vi "Measurement Logic.vi"() -> ()   [LabVIEW 2022 SP3, in "Stepped Frequency Sweep_Class D Amplifier.lvlib"]
uses:
  Stepped Frequency Sweep_Class D Amplifier.lvlib
  Measurement Results.ctl
  <vilib>/Analysis/NI_AALBase.lvlib
  <vilib>/Analysis/1siggen.llb/Ramp Pattern by Samples.vi
  <vilib>/Plug-In SDKs/Measurements/Measure Call Context/Measure Call Context.lvclass
  Measurement Configuration.ctl
  shared/controls/single tone audio measurements.ctl
  shared/controls/audio controls.lvlib
  shared/controls/weighting filter.ctl
  shared/controls/lowpass filter.ctl
  shared/controls/highpass filter.ctl
  shared/controls/sweep profile.ctl
  shared/controls/units - snr.ctl
  shared/controls/units - ratio.ctl
  shared/controls/digital output level units.ctl
  shared/controls/regulation target.ctl
  shared/controls/regulation target value units.ctl
panel:
  out "results":T1={"channel"="0", "frequency (Hz)"=1000.0000024177915, "amplitude (Vrms)"=-6.256665451281146, "amplitude (dBFS)"=78.42395339546047, "phase (deg)"=0.0, "SNR"=-71.07176133726693, "THD+N"=-71.98384642729017, "THD"=-0.25666545128114626, "dynamic range (dB)"=83.34902670182771, "gain"=102.93430172121762, "SFDR (dBc)"=0.0}
  out "Spectrum":cluster{"x0":dbl, "dx":dbl, "magnitude":dbl[]}(graph)
  out "Waveform Graph":waveform(dbl)(graph)
  out "measure call context out":refnum<class "Measure Call Context.lvclass">
  in  "measure call context in":refnum<class "Measure Call Context.lvclass">
  out "measurement results":T2={"channel name"="0", "frequency (Hz)"=[], "amplitude (Vrms)"=[], "amplitude (dBFS)"=[], "SNR"=[], "THD+N"=[], "THD"=[], "dynamic range (dB)"=[], "gain"=[], "SFDR (dBc)"=[], "output power (W)"=[], "wfm - t0"=0.0, "wfm - dt"=1.9531249997269942e-05, "wfm - data"=array[12800 elements], "fft - f0"=0.0, "fft - df"=4.000000000559116, "fft - data"=array[6400 elements]}
  in  "measurement configuration":T3={"digital serial cfg file"="", "digital channel list"="7821\\PCMo 8", "master clock channel list"="7821\\PCMo 0", "output level"=-10.0, "output level units"=enum."dBFS", "output range (pk-pk)"=15.0, "load impedance"=4.0, "signal phase"=0.0, "acq sampling rate"=51200.0, "min measurement cycles"=20, "min measurement time (s)"=0.1, "min settling cycles"=0, "min settling time (s)"=0.005, "acq channel"="PXI1Slot4/ai0", "band start"=20.0, "band stop"=20000.0, "weighting filter"=enum."Linear", "highpass filter"=enum."DC", "lowpass filter"=enum."No filter", "sweep start frequency (Hz)"=20.0, "sweep stop frequency (Hz)"=20000.0, "number of steps"=10, "sweep profile"=enum."Logarithmic", "SNR units"=enum."dB", "THD+N units"=enum."dB", "THD units"=enum."dB", "gain units"=enum."dB", "enable regulation"=FALSE, "regulation target"=enum."THD+N Ratio", "regulation target value"=10.0, "regulation target value units"=enum."%", "regulation start level"=-1.0, "regulation stop level"=-10.0, "regulation number of steps"=2} {"min measurement cycles" format="%#_6p"; "sweep stop frequency (Hz)" format="%0.2f"; "acq sampling rate" format="%0.2f"}
  out "error out":errorcluster
  in  "error in":errorcluster
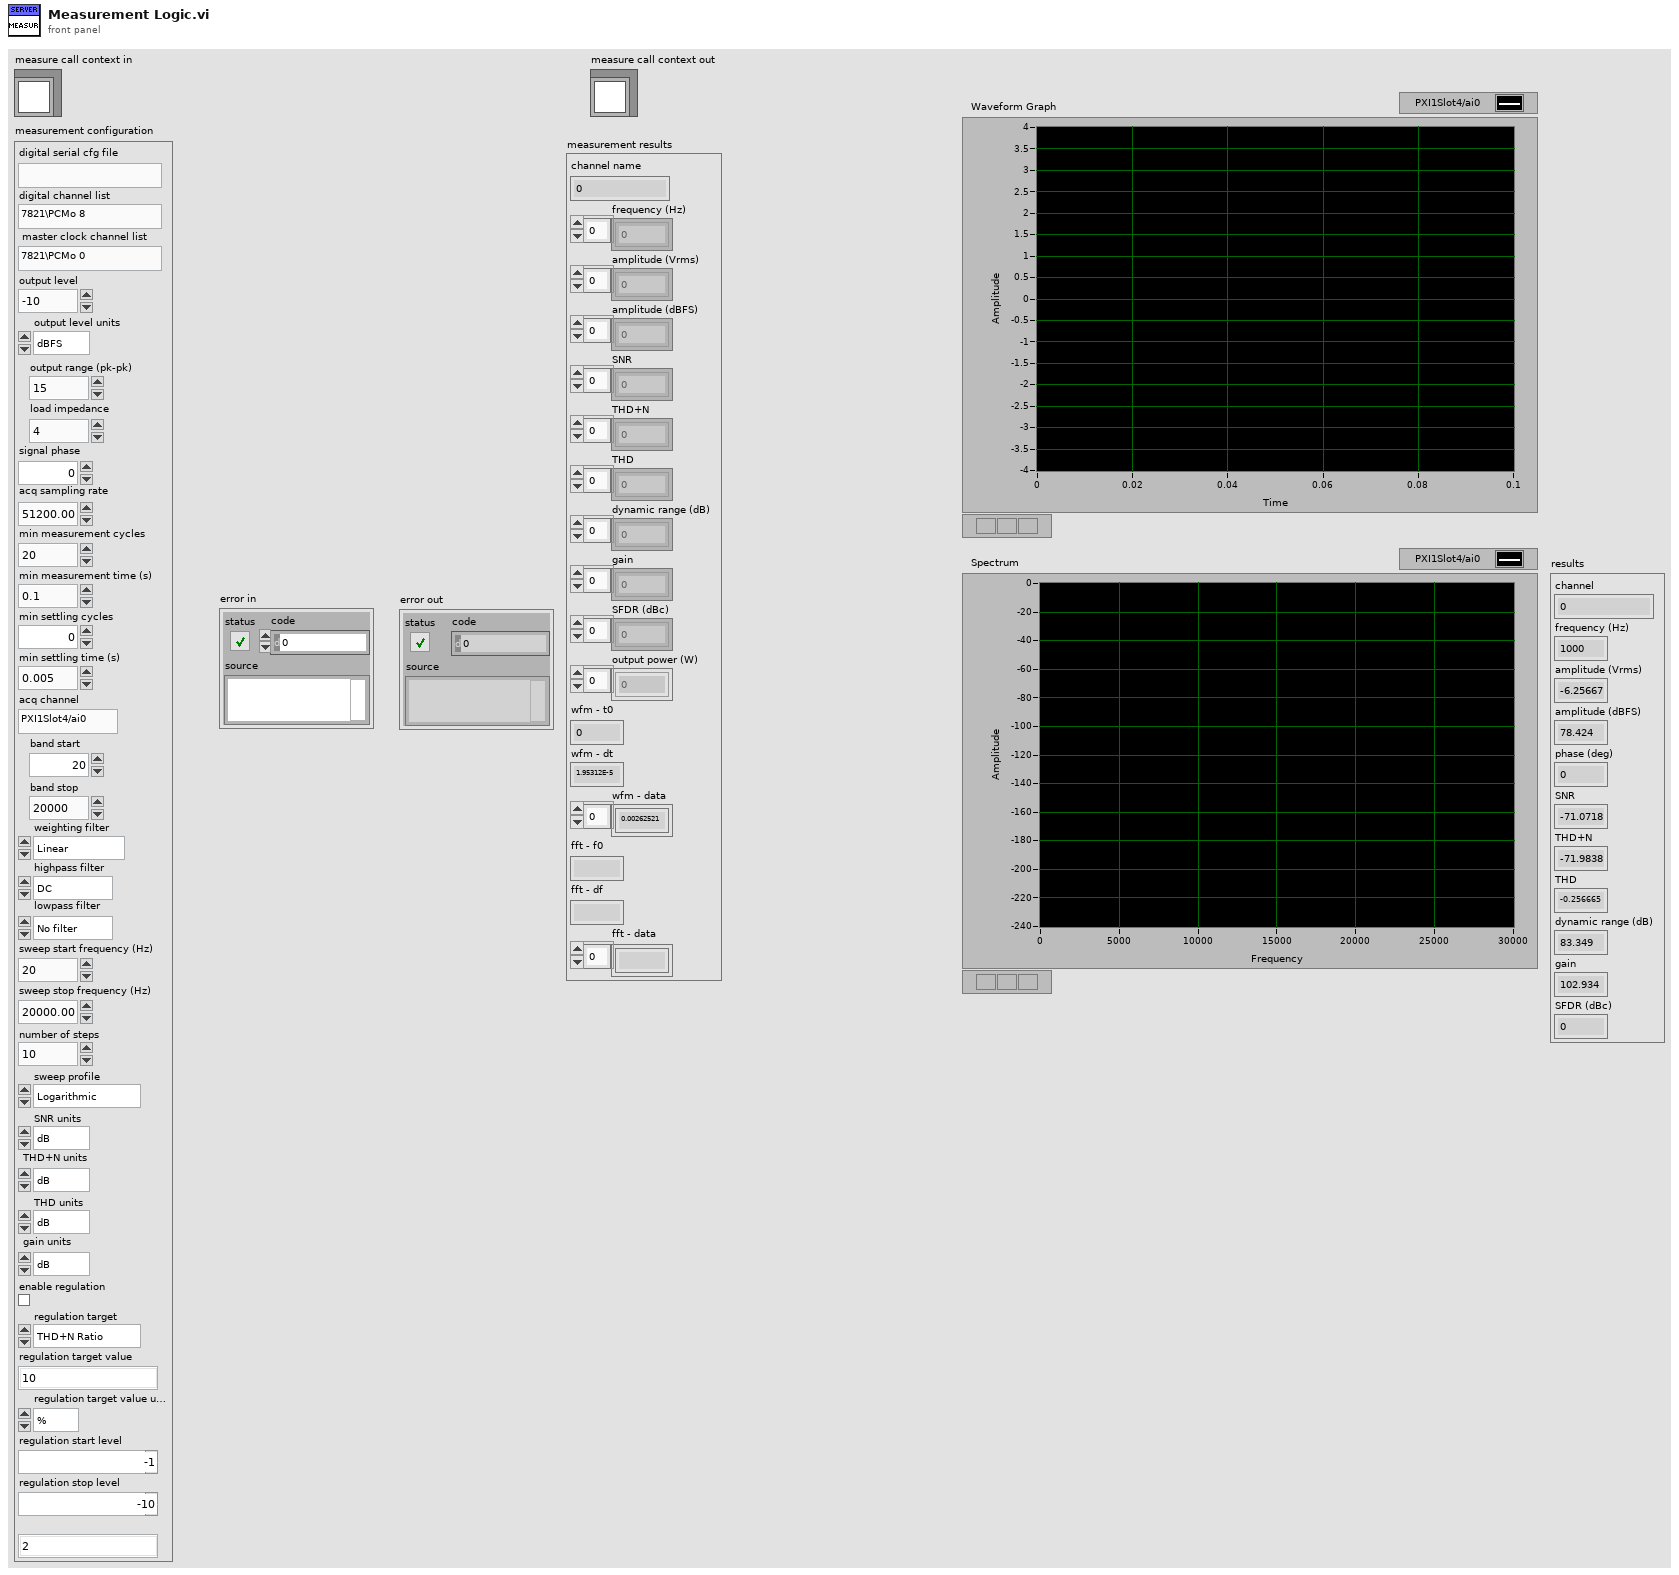
[diagram p1: front panel]
types:
  T1 = typedef "audio controls.lvlib/single tone audio measurements.ctl" = cluster{"channel":string, "frequency (Hz)":dbl, "amplitude (Vrms)":dbl, "amplitude (dBFS)":dbl, "phase (deg)":dbl, "SNR":dbl, "THD+N":dbl, "THD":dbl, "dynamic range (dB)":dbl, "gain":dbl, "SFDR (dBc)":dbl}
  T2 = typedef "Stepped Frequency Sweep_Class D Amplifier.lvlib/Measurement Results.ctl" = cluster{"channel name":string, "frequency (Hz)":dbl[], "amplitude (Vrms)":dbl[], "amplitude (dBFS)":dbl[], "SNR":dbl[], "THD+N":dbl[], "THD":dbl[], "dynamic range (dB)":dbl[], "gain":dbl[], "SFDR (dBc)":dbl[], "output power (W)":dbl[], "wfm - t0":dbl, "wfm - dt":dbl, "wfm - data":dbl[], "fft - f0":dbl, "fft - df":dbl, "fft - data":dbl[]}
  T3 = typedef "Stepped Frequency Sweep_Class D Amplifier.lvlib/Measurement Configuration.ctl" = cluster{"digital serial cfg file":string, "digital channel list":string, "master clock channel list":string, "output level":dbl, "output level units":T4, "output range (pk-pk)":dbl, "load impedance":dbl, "signal phase":dbl, "acq sampling rate":dbl, "min measurement cycles":u32, "min measurement time (s)":dbl, "min settling cycles":u32, "min settling time (s)":dbl, "acq channel":string, "band start":dbl, "band stop":dbl, "weighting filter":T5, "highpass filter":T6, "lowpass filter":T7, "sweep start frequency (Hz)":dbl, "sweep stop frequency (Hz)":dbl, "number of steps":u32, "sweep profile":T8, "SNR units":T9, "THD+N units":T10, "THD units":T10, "gain units":T10, "enable regulation":bool, "regulation target":T11, "regulation target value":dbl, "regulation target value units":T12, "regulation start level":dbl, "regulation stop level":dbl, "regulation number of steps":u32}
  T4 = typedef "audio controls.lvlib/digital output level units.ctl" = enum32{"% FS", "dBFS", "V"}
  T5 = typedef "weighting filter.ctl" = enum32{"Linear", "A-weighting", "B-weighting", "C-weighting"}
  T6 = typedef "highpass filter.ctl" = enum32{"DC", "AC"}
  T7 = typedef "lowpass filter.ctl" = enum32{"No filter", "AES17 20kHz", "AES17 40kHz"}
  T8 = typedef "audio controls.lvlib/sweep profile.ctl" = enum32{"Linear", "Logarithmic"}
  T9 = typedef "audio controls.lvlib/units - snr.ctl" = enum32{"dB", "x/y"}
  T10 = typedef "audio controls.lvlib/units - ratio.ctl" = enum32{"dB", "%", "x/y"}
  T11 = typedef "regulation target.ctl" = enum32{"THD+N Ratio", "Output Power"}
  T12 = typedef "regulation target value units.ctl" = enum32{"%", "W"}
  T13 = typedef "regulation settings.ctl" = cluster{"enable regulation":bool, "regulation target":T11, "regulation target value":dbl, "regulation target value units":T12, "regulation start level":dbl, "regulation stop level":dbl, "regulation number of steps":u32}
  T14 = typedef "single tone measurement settings (HW).ctl" = cluster{"digital channel list":string, "frame clock rate":dbl, "number of channels":u32, "channel length":u32, "bit depth":u32, "data justification":T15, "endianness":T16, "bit clock edge sync":T17, "frame sync edge for channel 0":T17, "channel 0 offset":u32, "master clock channel list":string, "master clock rate":dbl, "enable dither":bool, "logic level":T18, "signal frequency":dbl, "output level":dbl, "output level units":T4, "output range (pk-pk)":dbl, "load impedance":dbl, "signal phase":dbl, "acq sampling rate":dbl, "min measurement cycles":u32, "min measurement time (s)":dbl, "min settling cycles":u32, "min settling time (s)":dbl, "acq channel":string, "band start":dbl, "band stop":dbl, "weighting filter":T5, "highpass filter":T6, "lowpass filter":T7, "SNR units":T9, "THD+N units":T10, "THD units":T10, "gain units":T10}
  T15 = typedef "data justification.ctl" = enum32{"Left Justified", "Right Justified"}
  T16 = typedef "endianness.ctl" = enum32{"MSB First", "LSB First"}
  T17 = typedef "digital edge.ctl" = enum32{"Rising", "Falling"}
  T18 = typedef "logic level.ctl" = enum32{"3.3 V", "1.8 V", "1.2 V"}
  T19 = typedef "PCM tasks.ctl" = cluster{"PCM output task":T20, "PCM output task-clock":T20}
  T20 = typedef "PDM Acquisition Class Library.lvlib/PCM Output Task.lvclass/PCM Output Task DVR.ctl" = refnum<data-value>
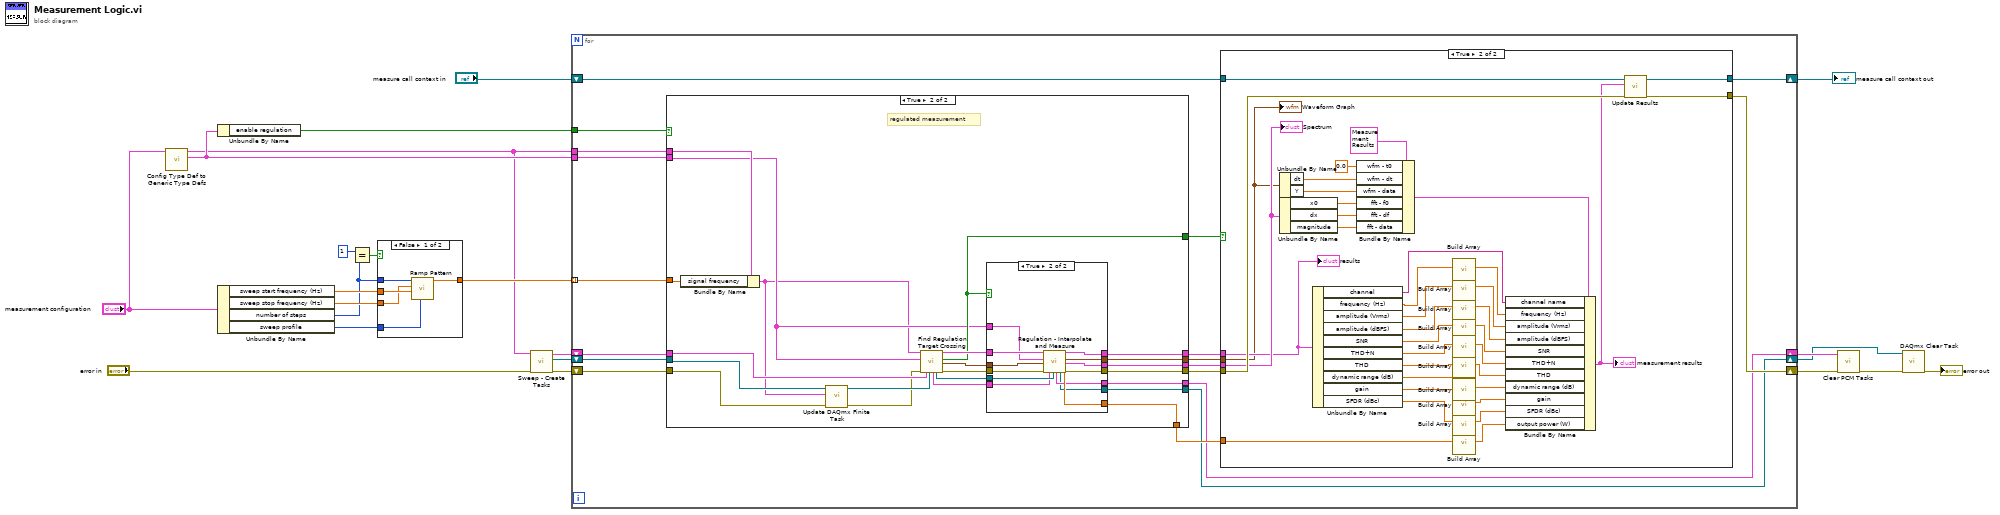
[diagram p0: block diagram]
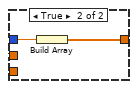
[diagram p2: hidden frame]
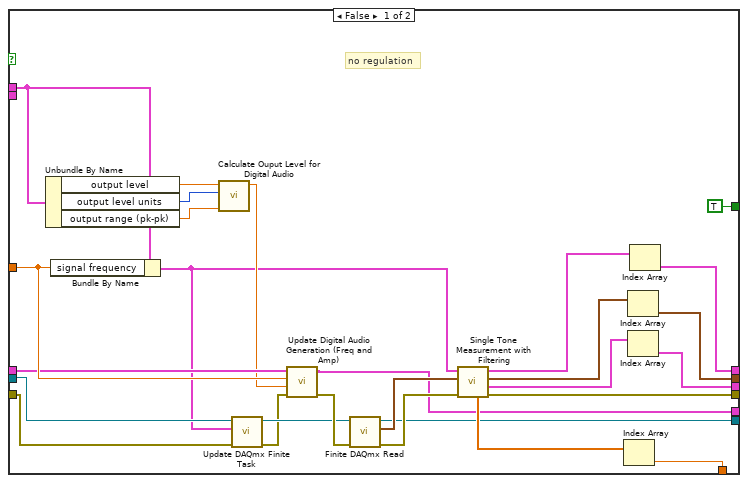
[diagram p4: hidden frame]
diagram:
  n1 = call "Config Type Def to Generic Type Defs.vi"("measurement configuration"="measurement configuration") -> ("regulation settings"=w11:T13, "single tone settings"=w8:T14)  [unwired: 9 in]
  n2 = Unbundle By Name(w11) -> ("enable regulation"=w13:bool)
  n3 = Unbundle By Name("measurement configuration") -> ("sweep start frequency (Hz)"=w21:dbl, "sweep stop frequency (Hz)"=w20:dbl, "number of steps"=w16:u32, "sweep profile"=w22:T8)
  n4 = Equal?(x=u32 1, y=w16) -> (x = y?=w17:bool)
  n5 = case shown="False" w17 {
    tunnel: w22 -> [w27 _]
    tunnel: w21 -> [w26 w29]
    tunnel: w20 -> [w25 _]
    tunnel: w16 -> [w24 _]
    tunnel: [w23 w28] -> w19
    frame False {
      n6 = call-poly <vilib>:"Ramp Pattern.vi"("type"=w27, "start"=w26, "end"=w25, "samples"=w24) -> ("Ramp Pattern"=w23:dbl[])  [unwired: 6 in, 1 out]
    }
    frame True {
      n7 = Build Array(w29) -> (w28:dbl[])
    }
  }
  n8 = call "Sweep - Create Tasks.vi"("error in (no error)"="error in", "measurement configuration"=w8) -> ("error out"=w10:errorcluster, "DAQmx task"=w7:refnum<k21>, "PCM tasks"=w2:T19)  [unwired: 7 in]
  n9 = for {
    tunnel: w19 -> [w39] mode=indexing
    shift-right: [w44] -> w6
    shift-left: w10 -> [w47]
    shift-right: [w45] -> w18
    shift-left: "measure call context in" -> [w43]
    tunnel: w13 -> [w38]
    tunnel: w8 -> [w35]
    tunnel: w11 -> [w34]
    shift-right: [w32] -> w3
    shift-left: w2 -> [w31]
    shift-right: [w30] -> w1
    shift-left: w7 -> [w33]
    n10 = case shown="True" w38 {
      tunnel: w47 -> [w88 w116]
      tunnel: [w100 w134] -> w46
      tunnel: [w111 w129] -> w42
      tunnel: [w110 w128] -> w41
      tunnel: [w109 w131] -> w40
      tunnel: w39 -> [w108 w126]
      tunnel: [w112 w130] -> w37
      tunnel: [TRUE ("crossing found?") w127] -> w36
      tunnel: w35 -> [w95 w125]
      tunnel: w34 -> [_ w124]
      tunnel: w31 -> [w106 w123]
      tunnel: w33 -> [w91 w118]
      tunnel: [w93 w119] -> w30
      tunnel: [w92 w120] -> w32
      frame False {
        # "no regulation"
        n11 = Unbundle By Name(w95) -> ("output level"=w98:dbl, "output level units"=w97:T4, "output range (pk-pk)"=w96:dbl)
        n12 = Bundle By Name(cluster=w95, "signal frequency"=w108) -> (w87:T14)
        n13 = call "Calculate Ouput Level for Digital Audio.vi"("output range (pk-pk)"=w96, "digital output level units"=w97, "output level"=w98) -> ("gain"=w94:dbl)  [unwired: 7 in, 1 out]
        n14 = call "Update DAQmx Finite Task.vi"("error in (no error)"=w88, "measurement configuration"=w87, "task/channels in"=w91) -> ("error out"=w89:errorcluster, "task out"=w90:refnum<k21>)  [unwired: 7 in]
        n15 = call "Update Digital Audio Generation (Freq and Amp).vi"("error in (no error)"=w89, "gain"=w94, "frequency"=w108, "PCM tasks"=w106) -> ("error out"=w107:errorcluster, "PCM tasks"=w92:T19)  [unwired: 6 in]
        n16 = call "Finite DAQmx Read.vi"("error in (no error)"=w107, "task/channels in"=w90) -> ("error out"=w105:errorcluster, "data"=w104:waveform(dbl)[], "task out"=w93:refnum<k21>)  [unwired: 7 in]
        n17 = call "Single Tone Measurement with Filtering.vi"("error in (no error)"=w105, "waveforms"=w104, "measurement configuration"=w87) -> ("error out"=w100:errorcluster, "spectra"=w101:cluster{"x0":dbl, "dx":dbl, "magnitude":dbl[]}[], "waveforms"=w102:waveform(dbl)[], "results"=w103:T1[], "output power"=w99:dbl[])  [unwired: 4 in]
        n18 = Index Array(array=w99) -> (element=w110:dbl)  [unwired: 1 in]
        n19 = Index Array(array=w102) -> (element=w112:waveform(dbl))  [unwired: 1 in]
        n20 = Index Array(array=w101) -> (element=w111:cluster{"x0":dbl, "dx":dbl, "magnitude":dbl[]})  [unwired: 1 in]
        n21 = Index Array(array=w103) -> (element=w109:T1)  [unwired: 1 in]
      }
      frame True {
        # "regulated measurement"
        n22 = Bundle By Name(cluster=w125, "signal frequency"=w126) -> (w114:T14)
        n23 = call "Update DAQmx Finite Task.vi"("error in (no error)"=w116, "measurement configuration"=w114, "task/channels in"=w118) -> ("error out"=w115:errorcluster, "task out"=w117:refnum<k21>)  [unwired: 7 in]
        n24 = call "Find Regulation Target Crossing.vi"("measurement configuration"=w114, "regaultion settings"=w124, "error in (no error)"=w115, "PCM tasks"=w123, "DAQmx task in"=w117) -> ("PCM tasks"=w121:T19, "DAQmx task out"=w122:refnum<k21>, "measurement configuration out"=w133:T14, "crossing found?"=w127:bool, "search results"=w132:cluster{"level":dbl, "value":dbl}[], "error out"=w135:errorcluster)  [unwired: 9 in]
        n25 = case shown="True" w127 {
          tunnel: w135 -> [w138 w150]
          tunnel: [w138 w148] -> w134
          tunnel: w133 -> [_ w151]
          tunnel: w132 -> [_ w149]
          tunnel: [_ w147] -> w131
          tunnel: [_ w146] -> w130
          tunnel: [_ w145] -> w129
          tunnel: [_ w144] -> w128
          tunnel: w124 -> [_ w143]
          tunnel: w122 -> [w137 w142]
          tunnel: w121 -> [w136 w141]
          tunnel: [w136 w140] -> w120
          tunnel: [w137 w139] -> w119
          frame False {
            # "could not regulate to value"
          }
          frame True {
            n26 = call "Regulation - Interpolate and Measure.vi"("measurement configuration"=w151, "regulation settings"=w143, "search results"=w149, "error in (no error)"=w150, "PCM tasks"=w141, "DAQmx task in"=w142) -> ("PCM tasks"=w140:T19, "DAQmx task out"=w139:refnum<k21>, "results"=w147:T1, "time domain"=w146:waveform(dbl), "spectrum"=w145:cluster{"x0":dbl, "dx":dbl, "magnitude":dbl[]}, "output power"=w144:dbl, "error out"=w148:errorcluster)  [unwired: 7 in]
          }
        }
      }
    }
    n27 = case shown="True" w36 {
      tunnel: w46 -> [w48 w86]
      tunnel: [w49 w85] -> w45
      tunnel: [w48 w84] -> w44
      tunnel: w43 -> [w49 w83]
      tunnel: w42 -> [_ w82]
      tunnel: w41 -> [_ w81]
      tunnel: w40 -> [_ w80]
      tunnel: w37 -> [_ w52]
      frame False {
        # "could not regulate, do not add measurement"
      }
      frame True {
        n28 = Unbundle By Name(w52) -> ("dt"=w51:dbl, "Y"=w50:dbl[])
        n29 = Unbundle By Name(w82) -> ("x0"=w78:dbl, "dx"=w77:dbl, "magnitude"=w76:dbl[])
        n30 = Unbundle By Name(w80) -> ("channel"=w53:string, "frequency (Hz)"=w54:dbl, "amplitude (Vrms)"=w55:dbl, "amplitude (dBFS)"=w56:dbl, "SNR"=w57:dbl, "THD+N"=w58:dbl, "THD"=w59:dbl, "dynamic range (dB)"=w60:dbl, "gain"=w61:dbl, "SFDR (dBc)"=w62:dbl)
        n31 = Bundle By Name(cluster=T2 {"channel name"="", "frequency (Hz)"=[], "amplitude (Vrms)"=[], "amplitude (dBFS)"=[], "SNR"=[], "THD+N"=[], "THD"=[], "dynamic range (dB)"=[], "gain"=[], "SFDR (dBc)"=[], "output power (W)"=[], "wfm - t0"=0.0, "wfm - dt"=0.0, "wfm - data"=[], "fft - f0"=0.0, "fft - df"=0.0, "fft - data"=[]} ("Measurement Results"), "wfm - t0"=0.0, "wfm - dt"=w51, "wfm - data"=w50, "fft - f0"=w78, "fft - df"=w77, "fft - data"=w76) -> (w74:T2)
        n32 = call "Build Array.vi"("value"=w54) -> ("Array"=w73:dbl[])  [unwired: 10 in]
        n33 = call "Build Array.vi"("value"=w55) -> ("Array"=w72:dbl[])  [unwired: 10 in]
        n34 = call "Build Array.vi"("value"=w56) -> ("Array"=w71:dbl[])  [unwired: 10 in]
        n35 = call "Build Array.vi"("value"=w57) -> ("Array"=w69:dbl[])  [unwired: 10 in]
        n36 = call "Build Array.vi"("value"=w58) -> ("Array"=w68:dbl[])  [unwired: 10 in]
        n37 = call "Build Array.vi"("value"=w59) -> ("Array"=w67:dbl[])  [unwired: 10 in]
        n38 = call "Build Array.vi"("value"=w60) -> ("Array"=w66:dbl[])  [unwired: 10 in]
        n39 = call "Build Array.vi"("value"=w61) -> ("Array"=w65:dbl[])  [unwired: 10 in]
        n40 = call "Build Array.vi"("value"=w62) -> ("Array"=w64:dbl[])  [unwired: 10 in]
        n41 = call "Build Array.vi"("value"=w81) -> ("Array"=w63:dbl[])  [unwired: 10 in]
        n42 = Bundle By Name(cluster=w74, "channel name"=w53, "frequency (Hz)"=w73, "amplitude (Vrms)"=w72, "amplitude (dBFS)"=w71, "SNR"=w69, "THD+N"=w68, "THD"=w67, "dynamic range (dB)"=w66, "gain"=w65, "SFDR (dBc)"=w64, "output power (W)"=w63) -> (w70:T2)
        "measurement results" <- w70
        n43 = call <vilib>:"Update Results.vi"("error in"=w86, "measurement results"=w70, "measure call context in"=w83) -> ("error out"=w84:errorcluster, "measure call context out"=w85:refnum<class "Measure Call Context.lvclass">)  [unwired: 7 in]
        "Waveform Graph" <- w52
        "Spectrum" <- w82
        "results" <- w80
      }
    }
  }
  "measure call context out" <- w18
  n44 = call "Clear PCM Tasks.vi"("error in (no error)"=w6, "PCM tasks"=w3) -> ("error out"=w5:errorcluster)  [unwired: 9 in]
  n45 = call <vilib>:"DAQmx Clear Task.vi"("task in"=w1, "error in"=w5) -> ("error out"=→"error out":errorcluster)  [unwired: 13 in]
